vi "县财政支持.vi"(7 "Radio Buttons":enum32{"Radio Selection 1", "Radio Selection 2"}(radio), 10 "Numeric":dbl, 11 "Combo Box":string(combo)) -> (9 "Boolean":bool)   [LabVIEW 2017]
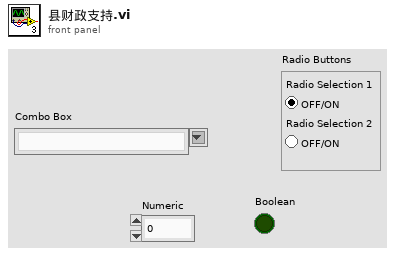
[diagram p1: front panel]
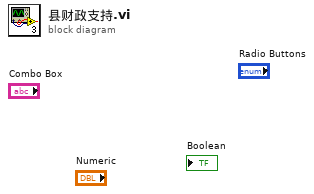
[diagram p0: block diagram]
diagram:
